vi "RemoteVI Menu Pointer.vi"(0 "write?":bool, 5 "state in":T1) -> (4 "state":T1)   [LabVIEW 2020, in "RemoteVI.lvlib"]
doc: "Keeps where the remote pointer is over the open LabVIEW popups and what the server did about it (docs\\architecture.md, Popups) - a functional global: a Feedback Node outside any loop, initialized on the first call only, so the state survives between calls of this non-reentrant VI (the composer builds no uninitialized shift register). With write? TRUE state in is stored; either way state is the stored value. Written by RemoteVI Note Popup Pointer.vi (pointer moves), RemoteVI Popup Click.vi (clicks), RemoteVI Swallow Button Up.vi and RemoteVI Menu Hover.vi (hover highlight and dwell, once per server loop iteration). Fields: active - a pointer position over the popups waits to be applied; x, y - that position in LOGICAL screen pixels; moved - tick count of the last pointer move; navigated - the position has been applied to the menu highlight; menu, top, hit - the menu window the highlight was last moved in, the top row of its highlight band (window pixels) and whether the band contains the pointer; row since - tick count since when that band is highlighted; dwelled - VK_RIGHT has been posted for this dwell; plain - a popup window that showed no highlight after VK_DOWN (colour picker, line width popup) and is operated with the mouse; swallow up - a button-down on a menu was turned into keys, so the matching button-up must not be posted. One server loop per LabVIEW instance, so one state is enough. Pure G, no I/O."
uses:
  RemoteVI.lvlib
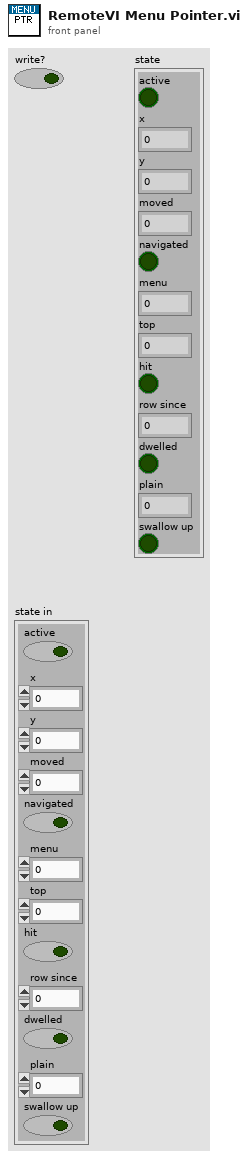
[diagram p1: front panel]
types:
  T1 = cluster{"active":bool, "x":i32, "y":i32, "moved":u32, "navigated":bool, "menu":u64, "top":i32, "hit":bool, "row since":u32, "dwelled":bool, "plain":u64, "swallow up":bool}
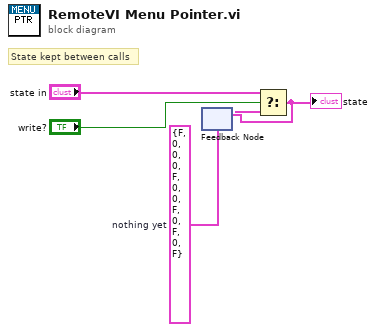
[diagram p0: block diagram]
diagram:
  w3 = T1 {"active"=FALSE, "x"=0, "y"=0, "moved"=0, "navigated"=FALSE, "menu"=0, "top"=0, "hit"=FALSE, "row since"=0, "dwelled"=FALSE, "plain"=0, "swallow up"=FALSE}  # nothing yet
  # "State kept between calls"
  n1 = feedback #1(w3) -> (w4:T1)
  n2 = Select(t="state in", s="write?", f=w4) -> (s? t:f=w5:T1)
  "state" <- w5
  n3 = feedback-in #1(w5) -> ()
